vi "create channels from assembly.vi"(8 "error in":errorcluster, 9 "assembly definition":T1, 10 "engine configuration in":refnum<class "engine configuration.lvclass">, 11 "EthernetIP configuration in":refnum<class "EthernetIP configuration.lvclass">) -> (0 "error out":errorcluster, 2 "engine configuration out":refnum<class "engine configuration.lvclass">, 3 "EthernetIP configuration out":refnum<class "EthernetIP configuration.lvclass">)   [LabVIEW 2013, in "EthernetIP editor node.lvclass"]
uses:
  EthernetIP editor node.lvclass
  configuration/assembly definition.ctl
  configuration/assembly type.ctl
  <vilib>/NI/Tag Bus/tag/Data Type.ctl
  <vilib>/NI/Module Execution Interface/Engine Configuration/engine configuration.lvclass
  configuration/EthernetIP configuration.lvclass
  configuration/EthernetIP configuration.lvclass/EthernetIP configuration.ctl
  <vilib>/NI/Configuration Framework/serializable configuration/NISE_CEF_serializable configuration.lvclass/NISE_CEF_serializable configuration.ctl
  channel/EthernetIP Channel.lvclass/EthernetIP Channel.ctl
  channel/Read Instance ID.vi
  channel/Read byte index.vi
  <vilib>/NI/Configuration Framework/serializable configuration/Read UID.vi
  configuration/read eip channels.vi
  configuration/Read assemblies.vi
  <vilib>/Utility/LVClass/Get LV Class Name.vi
  channel/EthernetIP Channel.lvclass
  <vilib>/NI/Tag Bus/tag/tag descriptor.lvclass
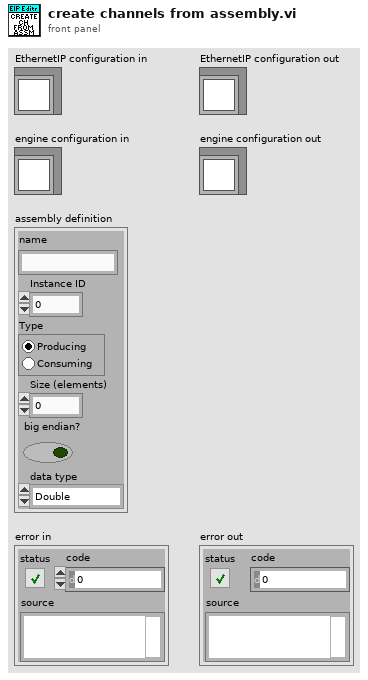
[diagram p1: front panel]
types:
  T1 = typedef "EthernetIP configuration.lvclass/assembly definition.ctl" = cluster{"name":string, "Instance ID":u32, "Type":T2, "Size (elements)":u32, "big endian?":bool, "data type":T3}
  T2 = typedef "EthernetIP configuration.lvclass/assembly type.ctl" = enum32{"Producing", "Consuming"}
  T3 = typedef "tag bus.lvlib/tag descriptor.lvclass/Data Type.ctl" = enum16{"Double", "Single", "I64", "I32", "I16", "I8", "U64", "U32", "U16", "U8", "Boolean", "String", "Array of Double", "Array of Single", "Array of I64", "Array of I32", "Array of I16", "Array of I8", "Array of U64", "Array of U32", "Array of U16", "Array of U8", "Array of Boolean", "Array of String"}
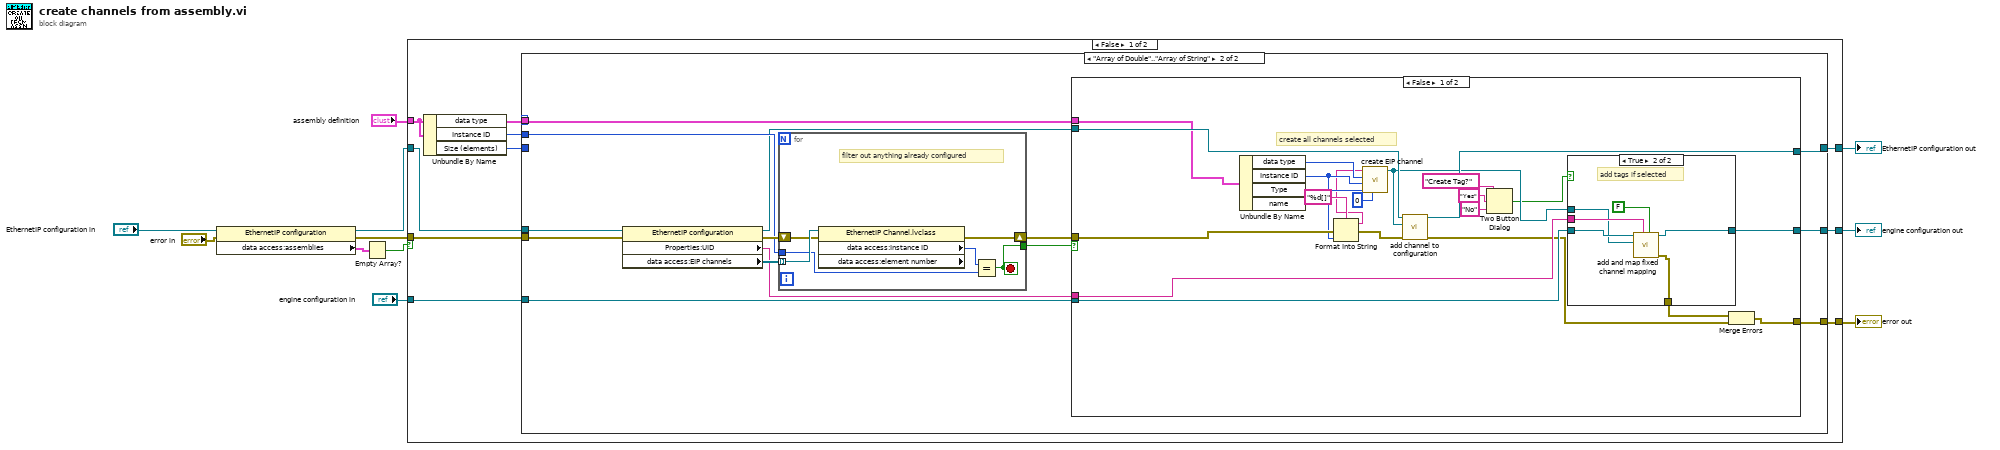
[diagram p0: block diagram]
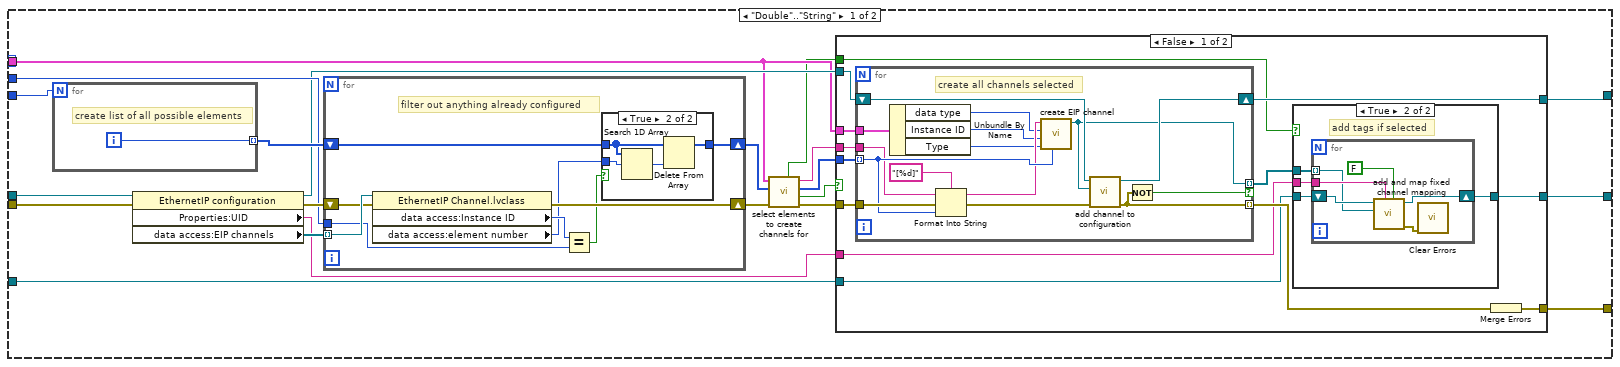
[diagram p2: hidden frame]
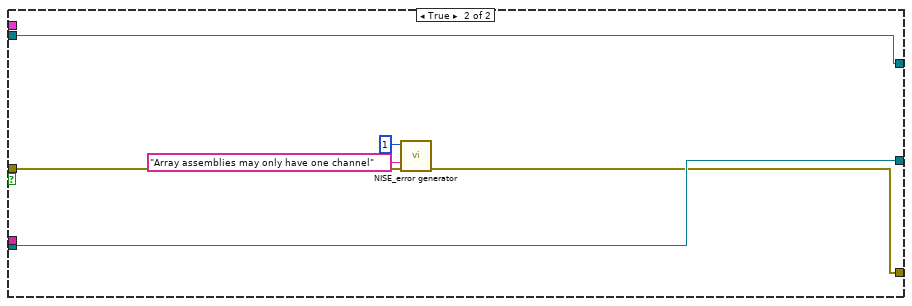
[diagram p7: hidden frame]
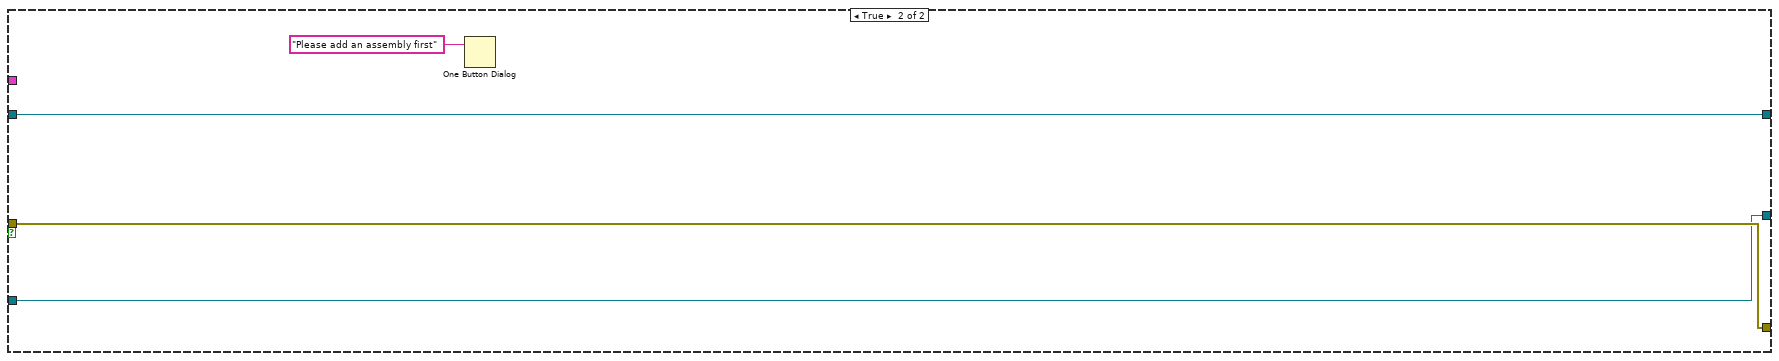
[diagram p8: hidden frame]
diagram:
  n1 = property class="EthernetIP configuration"(reference="EthernetIP configuration in", error in="error in") -> (reference out=w7:refnum<class "EthernetIP configuration.lvclass">, error out=w6:errorcluster, "data access:assemblies"=w9:T1[])
  n2 = Empty Array?(array=w9) -> (empty?=w8:bool)
  n3 = case shown="False" w8 {
    tunnel: w7 -> [w21 w158]
    tunnel: w6 -> [w20 w157]
    tunnel: [w17 w158] -> w5
    tunnel: [w16 w157] -> w4
    tunnel: "assembly definition" -> [w15 _]
    tunnel: [w14 w155] -> w1
    tunnel: "engine configuration in" -> [w13 w155]
    frame False {
      n4 = Unbundle By Name(w15) -> ("data type"=w12:T3, "Instance ID"=w18:u32, "Size (elements)"=w19:u32)
      n5 = case shown="\"Array of Double\"..\"Array of String\"" w12 {
        tunnel: w21 -> [w42 w113]
        tunnel: w20 -> [w41 w112]
        tunnel: w19 -> [w40 _]
        tunnel: w18 -> [w36 w109]
        tunnel: [w32 w107] -> w17
        tunnel: [w29 w105] -> w16
        tunnel: w15 -> [w26 w104]
        tunnel: [w24 w103] -> w14
        tunnel: w13 -> [w23 w102]
        frame "Double".."String" {
          n6 = for {
            N: w40 -> [_]
            tunnel: [w99] -> w39 mode=indexing
            i -> [w99]
            # "create list of all possible elements"
          }
          n7 = property class="EthernetIP configuration"(reference=w42, error in=w41) -> (reference out=w31:refnum<class "EthernetIP configuration.lvclass">, error out=w37:errorcluster, "Properties:UID"=w22:string, "data access:EIP channels"=w38:refnum<class "EthernetIP Channel.lvclass">[])
          n8 = for {
            shift-right: [w85] -> w34
            shift-left: w39 -> [w87]
            tunnel: w38 -> [w93] mode=indexing
            shift-right: [w91] -> w35
            shift-left: w37 -> [w92]
            tunnel: w36 -> [w89]
            # "filter out anything already configured"
            n9 = property class="EthernetIP Channel.lvclass"(reference=w93, error in=w92) -> (error out=w91:errorcluster, "data access:Instance ID"=w90:u32, "data access:element number"=w86:i32)  [unwired: 1 out]
            n10 = Equal?(x=w90, y=w89) -> (x = y?=w88:bool)
            n11 = case shown="True" w88 {
              tunnel: w87 -> [w94 w97]
              tunnel: w86 -> [_ w98]
              tunnel: [w94 w96] -> w85
              frame False {
              }
              frame True {
                n12 = Search 1D Array(1D array=w97, element=w98) -> (index of element=w95:i32)  [unwired: 1 in]
                n13 = Delete From Array(array=w97, index=w95) -> (array with subset deleted=w96:i32[])  [unwired: 1 in, 1 out]
              }
            }
          }
          n14 = call "select elements to create channels for.vi"("error in"=w35, "allowable channels"=w34, "assembly definition"=w26) -> ("error out"=w30:errorcluster, "cancelled?"=w33:bool, "channels to create"=w28:i32[], "base channame"=w27:string, "create tags"=w25:bool)  [unwired: 4 in]
          n15 = case shown="False" w33 {
            tunnel: [w52 w84] -> w32
            tunnel: w31 -> [w53 w84]
            tunnel: w30 -> [w55 w83]
            tunnel: [w49 w83] -> w29
            tunnel: w28 -> [w51 _]
            tunnel: w27 -> [w50 _]
            tunnel: w26 -> [w48 _]
            tunnel: w25 -> [w47 _]
            tunnel: [w46 w82] -> w24
            tunnel: w23 -> [w45 w82]
            tunnel: w22 -> [w44 _]
            frame False {
              n16 = for {
                shift-right: [w81] -> w52
                shift-left: w53 -> [w80]
                tunnel: w51 -> [w78] mode=indexing
                tunnel: w50 -> [w75]
                tunnel: w55 -> [w79]
                tunnel: [w68] -> w54 mode=indexing
                tunnel: w48 -> [w73]
                tunnel: [w69] -> w43 mode=indexing if=w67
                # "create all channels selected"
                n17 = Unbundle By Name(w73) -> ("data type"=w72:T3, "Instance ID"=w71:u32, "Type"=w70:T2)
                n18 = Format Into String(format string="[%d]", initial string=w75, error in=w79, w78) -> (resulting string=w74:string, error out=w77:errorcluster)
                n19 = call "create EIP channel.vi"("element"=w78, "Type"=w70, "Instance ID"=w71, "data type"=w72, "name"=w74) -> ("EthernetIP Channel out"=w69:refnum<class "EthernetIP Channel.lvclass">)  [unwired: 6 in]
                n20 = call "add channel to configuration.vi"("error in"=w77, "TBM channel in"=w69, "EthernetIP configuration in"=w80) -> ("error out"=w68:errorcluster, "EthernetIP configuration out"=w81:refnum<class "EthernetIP configuration.lvclass">)  [unwired: 7 in]
                n21 = Not(x=w68) -> (.not. x?=w67:bool)
              }
              n22 = case shown="True" w47 {
                tunnel: [w56 w59] -> w46
                tunnel: w45 -> [w56 w60]
                tunnel: w44 -> [_ w58]
                tunnel: w43 -> [_ w57]
                frame False {
                }
                frame True {
                  # "add tags if selected"
                  n23 = for {
                    shift-right: [w64] -> w59
                    shift-left: w60 -> [w66]
                    tunnel: w58 -> [w63]
                    tunnel: w57 -> [w61] mode=indexing
                    n24 = call <vilib>:"add and map fixed channel mapping.vi"("set module as owner"=FALSE, "module instance"=w63, "fixed channel"=w61, "engine configuration in"=w66) -> ("error out"=w65:errorcluster, "engine configuration out"=w64:refnum<class "engine configuration.lvclass">)  [unwired: 6 in]
                    n25 = call <vilib>:"Clear Errors.vi"("error in (no error)"=w65) -> ()  [unwired: 6 in, 1 out]
                  }
                }
              }
              n26 = Merge Errors(w54) -> (w49:errorcluster)
            }
            frame True {
            }
          }
        }
        frame "Array of Double".."Array of String" {
          n27 = property class="EthernetIP configuration"(reference=w113, error in=w112) -> (reference out=w106:refnum<class "EthernetIP configuration.lvclass">, error out=w110:errorcluster, "Properties:UID"=w101:string, "data access:EIP channels"=w111:refnum<class "EthernetIP Channel.lvclass">[])
          n28 = for {
            tunnel: w111 -> [w154] mode=indexing
            shift-right: [w152] -> w108
            shift-left: w110 -> [w153]
            tunnel: w109 -> [w150]
            tunnel: [w149] -> w100
            stop <- w149 stop-if-true
            # "filter out anything already configured"
            n29 = property class="EthernetIP Channel.lvclass" props=["data access:Instance ID", "data access:element number"](reference=w154, error in=w153) -> (error out=w152:errorcluster, "data access:Instance ID"=w151:u32)  [unwired: 2 out]
            n30 = Equal?(x=w151, y=w150) -> (x = y?=w149:bool)
          }
          n31 = case shown="False" w100 {
            tunnel: w108 -> [w128 w148]
            tunnel: [w135 w146] -> w107
            tunnel: w106 -> [w134 w146]
            tunnel: [w133 w145] -> w105
            tunnel: w104 -> [w132 _]
            tunnel: [w131 w147] -> w103
            tunnel: w102 -> [w130 w147]
            tunnel: w101 -> [w129 _]
            frame False {
              # "create all channels selected"
              n32 = Unbundle By Name(w132) -> ("data type"=w125:T3, "Instance ID"=w116:u32, "Type"=w124:T2)  [unwired: 1 out]
              n33 = Format Into String(format string="%d[]", error in=w128, w116) -> (resulting string=w114:string, error out=w117:errorcluster)  [unwired: 1 in]
              n34 = call "create EIP channel.vi"("element"=0, "Type"=w124, "Instance ID"=w116, "data type"=w125, "name"=w114) -> ("EthernetIP Channel out"=w126:refnum<class "EthernetIP Channel.lvclass">)  [unwired: 6 in]
              n35 = call "add channel to configuration.vi"("error in"=w117, "TBM channel in"=w126, "EthernetIP configuration in"=w134) -> ("error out"=w127:errorcluster, "EthernetIP configuration out"=w135:refnum<class "EthernetIP configuration.lvclass">)  [unwired: 7 in]
              n36 = Two Button Dialog(message="Create Tag?", 1:"No" ("F button name (\"Cancel\")"), 2:"Yes" ("T button name (\"OK\")")) -> (T button?=w120:bool)
              n37 = case shown="True" w120 {
                tunnel: [w136 w141] -> w131
                tunnel: w130 -> [w136 w142]
                tunnel: w129 -> [_ w140]
                tunnel: w126 -> [_ w139]
                tunnel: [_ w137] -> w118
                frame False {
                }
                frame True {
                  # "add tags if selected"
                  n38 = call <vilib>:"add and map fixed channel mapping.vi"("set module as owner"=FALSE, "module instance"=w140, "fixed channel"=w139, "engine configuration in"=w142) -> ("error out"=w137:errorcluster, "engine configuration out"=w141:refnum<class "engine configuration.lvclass">)  [unwired: 6 in]
                }
              }
              n39 = Merge Errors(w118, w127) -> (w133:errorcluster)
            }
            frame True {
              n40 = call <vilib>:"NISE_error generator.vi"("error in"=w148, "append error message"="Array assemblies may only have one channel", "error code (0)"=1) -> ("error out"=w145:errorcluster)  [unwired: 6 in]
            }
          }
        }
      }
    }
    frame True {
      n41 = One Button Dialog(message="Please add an assembly first") -> ()  [unwired: 1 in, 1 out]
    }
  }
  "engine configuration out" <- w1
  "EthernetIP configuration out" <- w5
  "error out" <- w4
